vi "VIH Project - Get Effective File Rule.vi"(5 "Don't Build Abs Paths (F)":bool, 6 "Ena <Invalid> (F)":bool, 7 "Ignore Control Rules (F)":bool, 8 "error in":errorcluster, 10 "File Path":path, 11 "Project Tree":T9) -> (0 "error out":errorcluster, 1 "Build Root Dir":path, 2 "Effective File Rule":T1, 3 "dup Project Tree":T9)   [LabVIEW 2014]
doc: "::: VI Helpeks :::\nCopyright (c) 2000-2026 Konstantin Shifershteyn. All rights reserved."
uses:
  VIH Project Tree Typedef - Tree Refnum.ctl
  _VIH HelpGen.llb/VIH HelpGen Typedef - Cluster - File Rule.ctl
  _VIH HelpGen.llb/VIH HelpGen Typedef - Enum - Default,Enable,Disable.ctl
  _VIH HelpGen.llb/VIH HelpGen Typedef - Cluster - File Rule - Source Paths.ctl
  _VIH HelpGen.llb/VIH HelpGen Typedef - Cluster - File Rule - Target Paths.ctl
  _VIH HelpGen.llb/VIH HelpGen Typedef - Enum - Description Mode.ctl
  _VIH HelpGen.llb/VIH HelpGen Typedef - Cluster - Control Rule.ctl
  _VIH HelpGen.llb/VIH HelpGen Typedef - Cluster - Enum Value Info.ctl
  _VIH HelpGen.llb/VIH HelpGen Typedef - Cluster - Group Rule - Flags.ctl
panel:
  # "VI Helpeks\nCopyright (c) 2012-2026 Konstantin Shifershteyn"
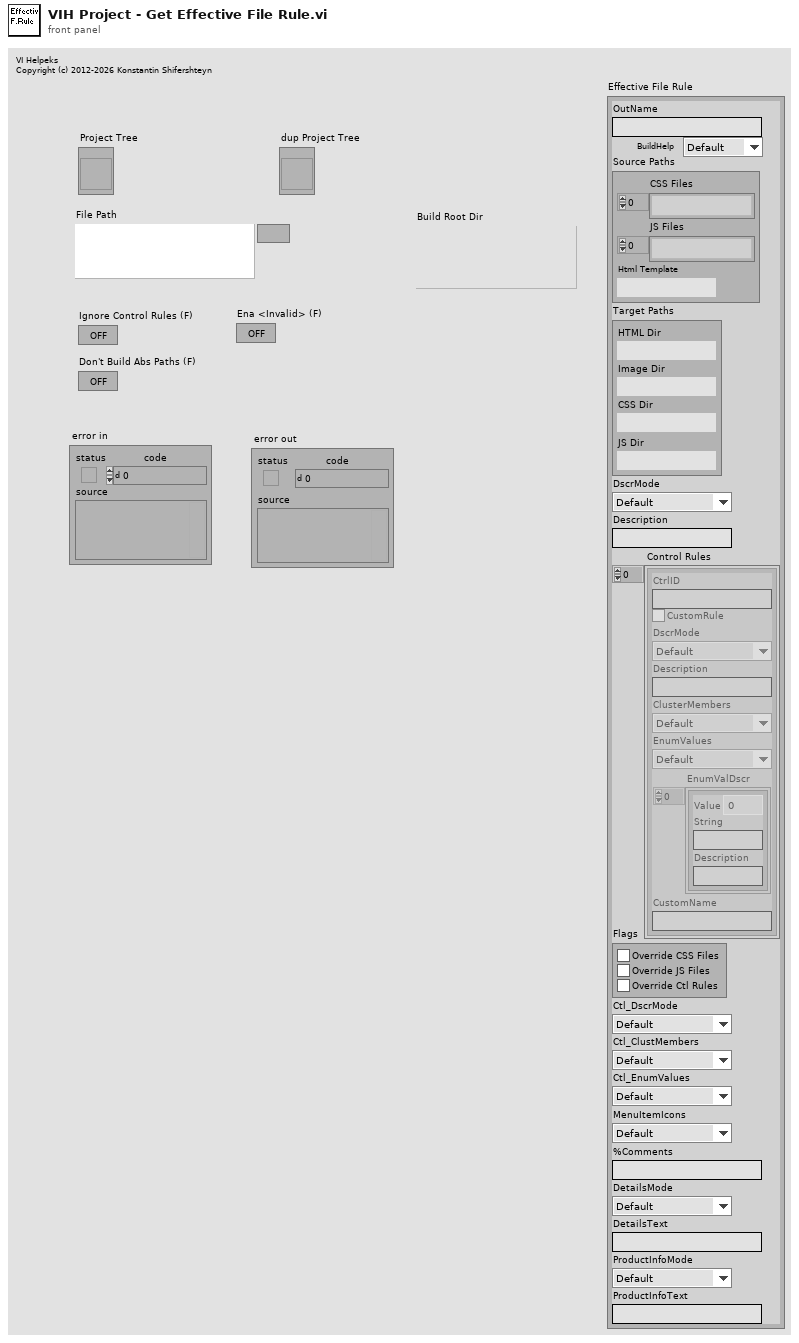
[diagram p1: front panel]
types:
  T1 = typedef "VIH HelpGen Typedef - Cluster - File Rule.ctl" = cluster{"OutName":string, "BuildHelp":T2, "Source Paths":T3, "Target Paths":T4, "DscrMode":T5, "Description":string, "Control Rules":T6[], "Flags":T8, "Ctl_DscrMode":T5, "Ctl_ClustMembers":T2, "Ctl_EnumValues":T2, "MenuItemIcons":T2, "%Comments":string, "DetailsMode":T5, "DetailsText":string, "ProductInfoMode":T2, "ProductInfoText":string}
  T2 = typedef "VIH HelpGen Typedef - Enum - Default,Enable,Disable.ctl" = enum16{"Default", "Enable", "Disable"}
  T3 = typedef "VIH HelpGen Typedef - Cluster - File Rule - Source Paths.ctl" = cluster{"CSS Files":path[], "JS Files":path[], "Html Template":path}
  T4 = typedef "VIH HelpGen Typedef - Cluster - File Rule - Target Paths.ctl" = cluster{"HTML Dir":path, "Image Dir":path, "CSS Dir":path, "JS Dir":path}
  T5 = typedef "VIH HelpGen Typedef - Enum - Description Mode.ctl" = enum16{"Default", "Description", "Description1", "Description2", "Custom", "None"}
  T6 = typedef "VIH HelpGen Typedef - Cluster - Control Rule.ctl" = cluster{"CtrlID":string, "CustomRule":bool, "DscrMode":T5, "Description":string, "ClusterMembers":T2, "EnumValues":T2, "EnumValDscr":T7[], "CustomName":string}
  T7 = typedef "VIH HelpGen Typedef - Cluster - Enum Value Info.ctl" = cluster{"Value":ext, "String":string, "Description":string}
  T8 = typedef "VIH HelpGen Typedef - Cluster - Group Rule - Flags.ctl" = cluster{"Override CSS Files":bool, "Override JS Files":bool, "Override Ctl Rules":bool}
  T9 = typedef "VIH Project Tree Typedef - Tree Refnum.ctl" = refnum<vi>
  T10 = typedef "VIH Project Tree Typedef - Tree Item Type.ctl" = enum32{"<Invalid>", "Project", "Proj Files", "Proj Rules", "File Group", "Rule Group", "Any File", "LV Func", ".mnu", ".mnu (dyn)", ".vi", ".vi (dyn)", ".vit", ".vit (dyn)", ".ctl", ".ctl (dyn)", ".ctt", ".ctt (dyn)", "polyVI", "polyVI (dyn)", "expVI", "expVI (dyn)", "HTML", "PolyVI Inst"}
  T11 = typedef "VIH HelpGen Typedef - Cluster - Group Rule.ctl" = cluster{"Source Root Dir":path, "Build Root Dir":path, "BuildHelp":T2, "Source Paths":T12, "Target Paths":T13, "VIDscrMode":T5, "MenuDscrMode":T5, "MenuItemIcons":T2, "Control Rules":T6[], "Flags":T8, "Ctl_DscrMode":T5, "Ctl_ClustMembers":T2, "Ctl_EnumValues":T2, "%Comments":string, "PVIIDscrMode":T5, "VIDetailsMode":T5, "ProductInfoMode":T2, "ProductInfoText":string}
  T12 = typedef "VIH HelpGen Typedef - Cluster - Group Rule - Source Paths.ctl" = cluster{"CSS Files":path[], "JS Files":path[], "VI Template":path, "Menu Template":path, "PolyVI Template":path}
  T13 = typedef "VIH HelpGen Typedef - Cluster - Group Rule - Target Paths.ctl" = cluster{"HTML Dir":path, "Image Dir":path, "CSS Dir":path, "JS Dir":path}
  T14 = typedef "VIH HelpGen Typedef - Palette - Item Type Enum.ctl" = enum32{"<Invalid>", "<unknown>", "VI", "Menu", "LV Func", "Express VI", "Poly VI", "CTL", "HTML"}
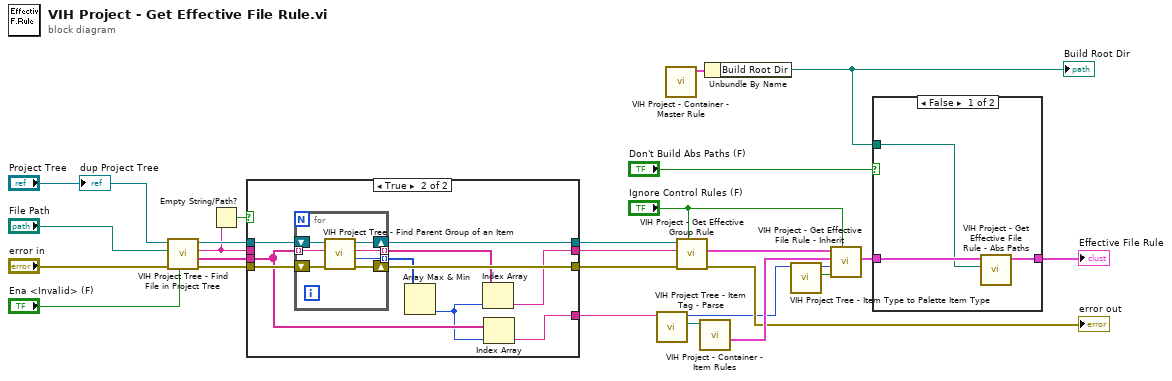
[diagram p0: block diagram]
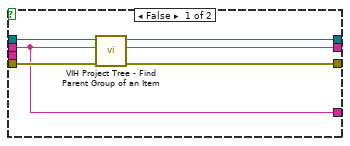
[diagram p2: hidden frame]
diagram:
  n1 = call "VIH Project Tree - Find File in Project Tree.vi"("Ena <Invalid> (F)"="Ena <Invalid> (F)", "error in"="error in", "File Path"="File Path", "Project Tree"="Project Tree") -> ("error out"=w16:errorcluster, "Tree Item Tags (Dynamic)"=w6:string[], "Tree Item Tag (Static)"=w9:string, "dup Project Tree"=w15:T9)  [unwired: 4 in]
  n2 = Empty String/Path?(string/path=w9) -> (empty?=w8:bool)
  n3 = case shown="True" w8 {
    tunnel: w16 -> [w32 w42]
    tunnel: w15 -> [w31 w41]
    tunnel: [w30 w40] -> w14
    tunnel: [w29 w39] -> w13
    tunnel: [w27 w35] -> w12
    tunnel: w9 -> [w28 _]
    tunnel: [w28 w36] -> w7
    tunnel: w6 -> [_ w37]
    frame False {
      n4 = call "VIH Project Tree - Find Parent Group of an Item.vi"("error in"=w32, "Tree Item Tag"=w28, "Project Tree"=w31) -> ("error out"=w29:errorcluster, "Parent Group Tag"=w27:string, "dup Project Tree"=w30:T9)  [unwired: 5 in, 1 out]
    }
    frame True {
      n5 = for {
        shift-right: [w46] -> w39
        shift-left: w42 -> [w49]
        shift-right: [w47] -> w40
        shift-left: w41 -> [w48]
        tunnel: w37 -> [w45] mode=indexing
        tunnel: [w44] -> w38 mode=indexing
        tunnel: [w43] -> w34 mode=indexing
        n6 = call "VIH Project Tree - Find Parent Group of an Item.vi"("error in"=w49, "Tree Item Tag"=w45, "Project Tree"=w48) -> ("error out"=w46:errorcluster, "Level"=w43:i32, "Parent Group Tag"=w44:string, "dup Project Tree"=w47:T9)  [unwired: 5 in]
      }
      n7 = Array Max & Min(array=w34) -> (min index (indices)=w33:i32)  [unwired: 3 out]
      n8 = Index Array(array=w38, index=w33) -> (element=w35:string)
      n9 = Index Array(array=w37, index=w33) -> (element=w36:string)
    }
  }
  n10 = call "VIH Project Tree - Item Tag - Parse.vi"("Tree Item Tag"=w7) -> ("Item File Path"=w3:path, "Item Type"=w11:T10)  [unwired: 8 in, 1 out]
  n11 = call "VIH Project - Container - Master Rule.vi"() -> ("Rule out"=w5:T11)  [unwired: 11 in]
  n12 = call "VIH Project - Get Effective Group Rule.vi"("Ignore Control Rules (F)"="Ignore Control Rules (F)", "error in"=w13, "Group ID"=w12, "Project Tree"=w14) -> ("error out"=→"error out":errorcluster, "Effective Group Rule"=w23:T11)  [unwired: 5 in, 1 out]
  n13 = call "VIH Project - Container - Item Rules.vi"("Item Path"=w3) -> ("Item Rule out"=w22:T1)  [unwired: 6 in, 4 out]
  n14 = Unbundle By Name(w5) -> ("Build Root Dir"=w4:path)
  "Build Root Dir" <- w4
  n15 = call "VIH Project Tree - Item Type to Palette Item Type.vi"("Tree Item Type"=w11) -> ("PolyVI Instance VI"=w2:bool, "Item/File Type"=w10:T14)  [unwired: 9 in]
  n16 = call "VIH Project - Get Effective File Rule - Inherit.vi"("Ignore Control Rules (F)"="Ignore Control Rules (F)", "PolyVI Instance VI"=w2, "File Type"=w10, "File Rule"=w22, "Parent Group Rule"=w23) -> ("Effective File Rule"=w19:T1)  [unwired: 6 in]
  n17 = case shown="False" "Don't Build Abs Paths (F)" {
    tunnel: w19 -> [w52 w53]
    tunnel: [w51 w53] -> w18
    tunnel: w4 -> [w50 _]
    frame False {
      n18 = call "VIH Project - Get Effective File Rule - Abs Paths.vi"("Build Root Dir"=w50, "File Rule in"=w52) -> ("File Rule out"=w51:T1)  [unwired: 9 in]
    }
    frame True {
    }
  }
  "Effective File Rule" <- w18
  "dup Project Tree" <- "Project Tree"
